vi "Cleanup.vi"(8 "error in (no error)":errorcluster, 11 "2DArrayManager in":refnum<class "2DArrayManager.lvclass">) -> (0 "error out":errorcluster)   [LabVIEW 2020, in "OOPanel.lvlib" / "2DArrayManager.lvclass"]
uses:
  2DArrayManager.lvclass
  2DArrayManager.lvclass/2DArrayManager.ctl
  Manager/Manager.lvclass
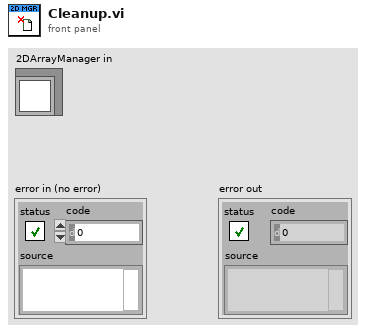
[diagram p1: front panel]
types:
  T1 = typedef "OOPanel.lvlib/2DArrayManager.lvclass/Events.ctl" = cluster{"Stop":refnum<user-event>, "Update":refnum<user-event>, "Set BG":refnum<user-event>, "Scroll":refnum<user-event>, "Highlight":refnum<user-event>, "Synced Scroll":refnum<user-event>, "Scrollbars":refnum<user-event>}
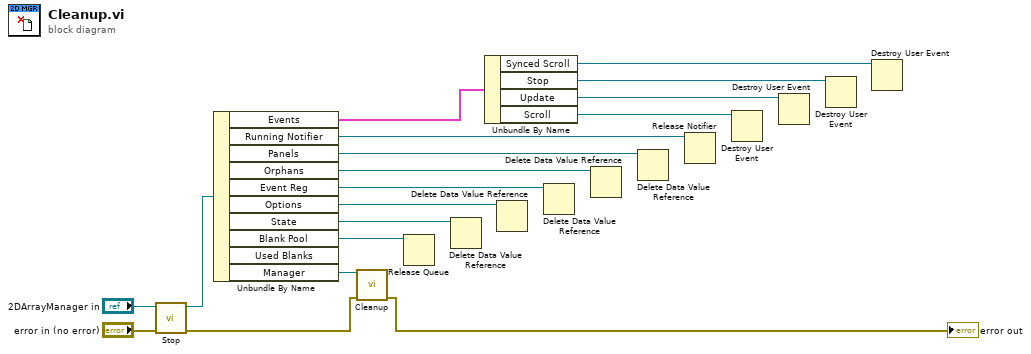
[diagram p0: block diagram]
diagram:
  n1 = call "Stop.vi"("error in (no error)"="error in (no error)", "2DArrayManager in"="2DArrayManager in") -> ("error out"=w2:errorcluster, "2DArrayManager out"=w16:refnum<class "2DArrayManager.lvclass">)  [unwired: 8 in]
  n2 = Unbundle By Name(w16) -> ("Events"=w10:T1, "Running Notifier"=w11:refnum<notifier>, "Panels"=w12:refnum<data-value>, "Orphans"=w13:refnum<data-value>, "Event Reg"=w14:refnum<data-value>, "Options"=w15:refnum<data-value>, "State"=w5:refnum<data-value>, "Blank Pool"=w4:refnum<queue>, "Manager"=w3:refnum<class "Manager.lvclass">)  [unwired: 1 out]
  n3 = call "Cleanup.vi"("error in (no error)"=w2, "Manager in"=w3) -> ("error out"=→"error out":errorcluster)  [unwired: 7 in, 2 out]
  n4 = Release Queue(queue=w4) -> ()  [unwired: 2 in, 3 out]
  n5 = Delete Data Value Reference(data value reference=w5) -> ()  [unwired: 1 in, 2 out]
  n6 = Unbundle By Name(w10) -> ("Synced Scroll"=w6:refnum<user-event>, "Stop"=w7:refnum<user-event>, "Update"=w8:refnum<user-event>, "Scroll"=w9:refnum<user-event>)
  n7 = Delete Data Value Reference(data value reference=w15) -> ()  [unwired: 1 in, 2 out]
  n8 = Delete Data Value Reference(data value reference=w14) -> ()  [unwired: 1 in, 2 out]
  n9 = Delete Data Value Reference(data value reference=w13) -> ()  [unwired: 1 in, 2 out]
  n10 = Delete Data Value Reference(data value reference=w12) -> ()  [unwired: 1 in, 2 out]
  n11 = Release Notifier(notifier=w11) -> ()  [unwired: 2 in, 3 out]
  n12 = Destroy User Event(user event=w9) -> ()  [unwired: 1 in, 1 out]
  n13 = Destroy User Event(user event=w8) -> ()  [unwired: 1 in, 1 out]
  n14 = Destroy User Event(user event=w7) -> ()  [unwired: 1 in, 1 out]
  n15 = Destroy User Event(user event=w6) -> ()  [unwired: 1 in, 1 out]
